vi "Element Init.vi"(7 "VolatusAPI":refnum<class "VolatusAPI.lvclass">, 8 "error in (no error)":errorcluster, 10 "JSON":string, 11 "LoggingControl in":refnum<class "GroupLoggingControl.lvclass">) -> (0 "error out":errorcluster, 3 "LoggingControl out":refnum<class "GroupLoggingControl.lvclass">)   [LabVIEW 2020, in "VolatusGUIElements.lvlib" / "GroupLoggingControl.lvclass"]
uses:
  GroupLoggingControl.lvclass
  C:/dev/lv20CE/relink/lv-volatus/VolatusGUI/GUI Element/GUI Element.lvclass
  Volatus/VolatusAPI/VolatusAPI.lvclass
  JSON.ctl
  Prompt Result.ctl
  Prompt Action.ctl
  VolatusGUI/GUI Element/GUI Element.lvclass/GUI Element.ctl
  GroupLoggingControl.lvclass/GroupLoggingControl.ctl
  6b4406ff-dbb0-478f-9794-4f2464f74e8d.vi
  <vilib>/JDP Science/JSONtext/JSON text to Variant.vi
  <vilib>/JDP Science/JSONtext/LVClass Serializer/JSONtext LVClass Serializer.lvclass
  VolatusGUI/GUI Element/GUI Element.lvclass
  Log Group Status.ctl
  Command Info.ctl
  Log Group.ctl
  Target Info.ctl
  Status.ctl
  C:/dev/lv20CE/relink/lv-volatus/VolatusGUIElements/GroupLoggingControl/GroupLoggingControl.lvclass
  C:/dev/lv20CE/relink/lv-volatus/VolatusGUI/OnValueChangeHandler/OnValueChangeHandler.lvclass
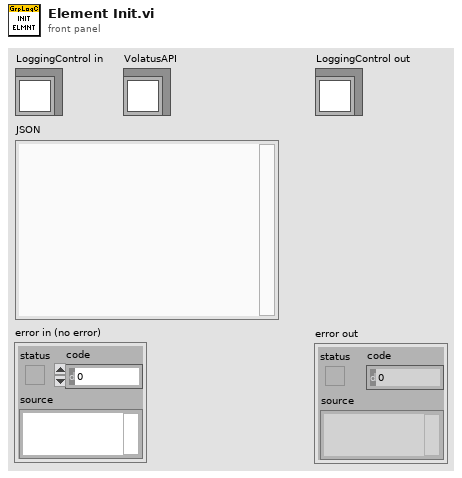
[diagram p1: front panel]
types:
  T1 = typedef "VolatusGUIElements.lvlib/GroupLoggingControl.lvclass/Status.ctl" = cluster{"Groups":T2[], "Targets":T5[]}
  T2 = typedef "VolatusGUIElements.lvlib/GroupLoggingControl.lvclass/Log Group.ctl" = cluster{"Status":T3, "Command Info":T4, "Logging":bool, "State":string}
  T3 = typedef "VolatusGUIElements.lvlib/GroupLoggingControl.lvclass/Log Group Status.ctl" = cluster{"Group":string, "Group Color":u32, "Button":bool}
  T4 = typedef "VolatusGUIElements.lvlib/GroupLoggingControl.lvclass/Command Info.ctl" = cluster{"Commanding":bool, "Cmd Time":dbl, "Group ID":string}
  T5 = typedef "VolatusGUIElements.lvlib/GroupLoggingControl.lvclass/Target Info.ctl" = cluster{"Node":string, "Node Color":u32, "Groups":T2[]}
  T6 = typedef "VolatusGUIElements.lvlib/GroupLoggingControl.lvclass/Prompt Result.ctl" = cluster{"Action":T7, "Series":string, "Timestamp":string, "Target (All)":string, "Group (All)":string}
  T7 = typedef "VolatusGUIElements.lvlib/GroupLoggingControl.lvclass/Prompt Action.ctl" = enum16{"Cancelled", "Started"}
  T8 = typedef "VolatusGUIElements.lvlib/GroupLoggingControl.lvclass/JSON.ctl" = cluster{"Groups":cluster{"Label":string, "Group":string}[], "Targets":cluster{"Node":string, "Groups":cluster{"Label":string, "Group":string}[]}[]}
  T9 = cluster{"Node":string, "Groups":cluster{"Label":string, "Group":string}[]}[]
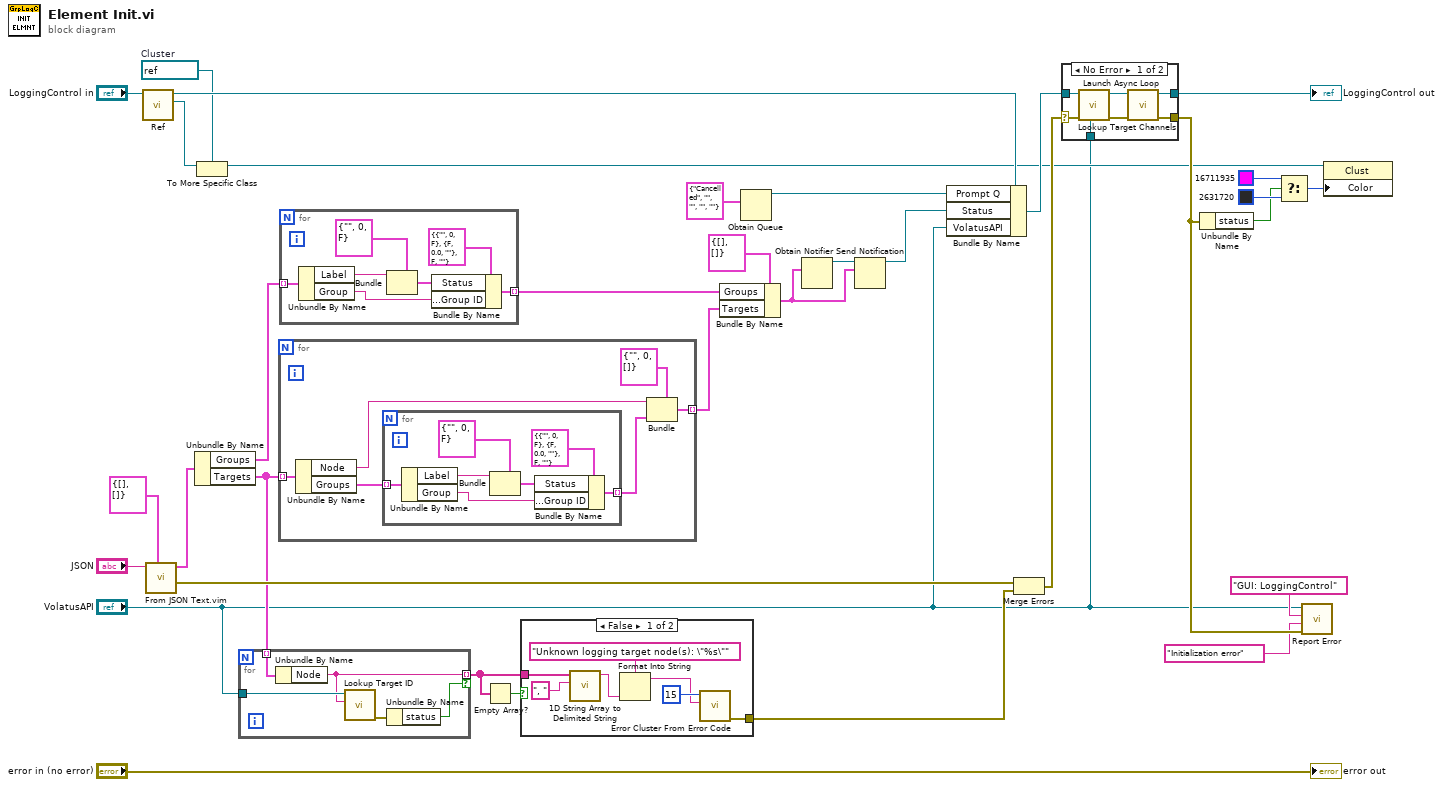
[diagram p0: block diagram]
diagram:
  w12 = refnum<vi> refnum  # Cluster
  n1 = call "Ref.vi"("GUI Element in"="LoggingControl in") -> ("Ref"=w13:refnum<vi>, "GUI Element out"=w14:refnum<class "GroupLoggingControl.lvclass">)  [unwired: 9 in]
  n2 = call "From JSON Text.vim"("Data Type and Default Value"=T8 {"Groups"=[], "Targets"=[]} ("JSON"), "JSON"="JSON") -> ("error out"=w28:errorcluster, "Data out"=w29:T8)  [unwired: 8 in]
  n3 = Unbundle By Name(w29) -> ("Groups"=w7:cluster{"Label":string, "Group":string}[], "Targets"=w9:T9)
  n4 = To More Specific Class(target class=w12, reference=w13) -> (specific class reference=w11:refnum<vi>)  [unwired: 1 in, 1 out]
  n5 = for {
    tunnel: "VolatusAPI" -> [w39]
    tunnel: w9 -> [w36] mode=indexing
    tunnel: [w35] -> w26 mode=indexing if=w37
    n6 = Unbundle By Name(w36) -> ("Node"=w35:string)
    n7 = call "Lookup Target ID.vi"("Target Name"=w35, "VolatusAPI in"=w39) -> ("error out"=w38:errorcluster)  [unwired: 6 in, 3 out]
    n8 = Unbundle By Name(w38) -> ("status"=w37:bool)
  }
  n9 = for {
    tunnel: w9 -> [w45] mode=indexing
    tunnel: [w40] -> w3 mode=indexing
    n10 = Unbundle By Name(w45) -> ("Node"=w44:string, "Groups"=w42:cluster{"Label":string, "Group":string}[])
    n11 = for {
      tunnel: w42 -> [w52] mode=indexing
      tunnel: [w47] -> w41 mode=indexing
      n12 = Unbundle By Name(w52) -> ("Label"=w51:string, "Group"=w46:string)
      n13 = Bundle(cluster=T3 {"Group"="", "Group Color"=0, "Button"=FALSE} ("Log Group Status"), "Group"=w51) -> (w48:T3)  [unwired: 2 in]
      n14 = Bundle By Name(cluster=T2 {"Status"={"Group"="", "Group Color"=0, "Button"=FALSE}, "Command Info"={"Commanding"=FALSE, "Cmd Time"=0.0, "Group ID"=""}, "Logging"=FALSE, "State"=""} ("Log Group"), "Status"=w48, "Command Info.Group ID"=w46) -> (w47:T2)
    }
    n15 = Bundle(cluster=T5 {"Node"="", "Node Color"=0, "Groups"=[]} ("Node Info"), "Node"=w44, "Groups"=w41) -> (w40:T5)  [unwired: 1 in]
  }
  n16 = for {
    tunnel: w7 -> [w59] mode=indexing
    tunnel: [w54] -> w6 mode=indexing
    n17 = Unbundle By Name(w59) -> ("Label"=w58:string, "Group"=w53:string)
    n18 = Bundle(cluster=T3 {"Group"="", "Group Color"=0, "Button"=FALSE} ("Log Group Status"), "Group"=w58) -> (w55:T3)  [unwired: 2 in]
    n19 = Bundle By Name(cluster=T2 {"Status"={"Group"="", "Group Color"=0, "Button"=FALSE}, "Command Info"={"Commanding"=FALSE, "Cmd Time"=0.0, "Group ID"=""}, "Logging"=FALSE, "State"=""} ("Log Group"), "Status"=w55, "Command Info.Group ID"=w53) -> (w54:T2)
  }
  n20 = Empty Array?(array=w26) -> (empty?=w27:bool)
  n21 = case shown="False" w27 {
    tunnel: w26 -> [w66 _]
    tunnel: [w60 _] -> w25
    frame False {
      n22 = call <vilib>:"1D String Array to Delimited String.vi"("delimiter"=", ", "string array"=w66) -> ("delimited string"=w63:string)  [unwired: 9 in]
      n23 = Format Into String(format string="Unknown logging target node(s): \"%s\"", w63) -> (resulting string=w61:string)  [unwired: 2 in, 1 out]
      n24 = call <vilib>:"Error Cluster From Error Code.vi"("error message (\"\")"=w61, "error code (0)"=15) -> ("error out"=w60:errorcluster)  [unwired: 7 in]
    }
    frame True {
    }
  }
  n25 = Bundle By Name(cluster=T1 {"Groups"=[], "Targets"=[]} ("Status"), "Groups"=w6, "Targets"=w3) -> (w2:T1)
  n26 = Obtain Queue(element data type=T6 {"Action"=enum."Cancelled", "Series"="", "Timestamp"="", "Target (All)"="", "Group (All)"=""} ("Prompt Result")) -> (queue out=w15:refnum<queue>)  [unwired: 4 in, 2 out]
  n27 = Obtain Notifier(notification data type=w2) -> (notifier out=w4:refnum<notifier>)  [unwired: 3 in, 2 out]
  n28 = Send Notification(notification=w2, notifier=w4) -> (notifier out=w1:refnum<notifier>)  [unwired: 1 in, 1 out]
  n29 = Bundle By Name(cluster=w14, "Prompt Q"=w15, "Status"=w1, "VolatusAPI"="VolatusAPI") -> (w32:refnum<class "GroupLoggingControl.lvclass">)
  n30 = Merge Errors(w28, w25) -> (w17:errorcluster)
  n31 = case shown="No Error" w17 {
    selector: w17 -> [w72 w75]
    tunnel: w32 -> [w73 w74]
    tunnel: [w67 w74] -> w18
    tunnel: [w69 w75] -> w34
    tunnel: "VolatusAPI" -> [w70 _]
    frame No Error {
      n32 = call "Lookup Target Channels.vi"("VolatusAPI"=w70, "error in (no error)"=w72, "LoggingControl in"=w73) -> ("error out"=w71:errorcluster, "LoggingControl out"=w68:refnum<class "GroupLoggingControl.lvclass">)  [unwired: 7 in]
      n33 = call "Launch Async Loop.vi"("error in (no error)"=w71, "GroupLoggingControl in"=w68) -> ("error out"=w69:errorcluster, "GroupLoggingControl out"=w67:refnum<class "GroupLoggingControl.lvclass">)  [unwired: 8 in]
    }
    frame Error {
    }
  }
  "LoggingControl out" <- w18
  n34 = Unbundle By Name(w34) -> ("status"=w20:bool)
  n35 = Select(t=u32 16711935 ("Color"), s=w20, f=u32 2631720 ("Color")) -> (s? t:f=w21:u32)
  n36 = call "Report Error.vi"("error in (no error)"=w34, "Message"="Initialization error", "Context"="GUI: LoggingControl", "VolatusAPI in"="VolatusAPI") -> ()  [unwired: 6 in, 2 out]
  n37 = property class="Clust"(reference=w11, "Color"=w21) -> ()  [unwired: 1 in, 2 out]
  "error out" <- "error in (no error)"
